vi "close.vi"(8 "error in":errorcluster, 11 "Scan Engine runtime in":refnum<class "Scan Engine runtime.lvclass">) -> (0 "error out":errorcluster)   [LabVIEW 2015, in "Scan Engine runtime.lvclass"]
doc: "Provides an interface for terminating a module instance. While this interface performs no operations, a child should close and deallocate any open references or memory."
uses:
  Scan Engine runtime.lvclass
  Scan Engine runtime.lvclass/Scan Engine runtime.ctl
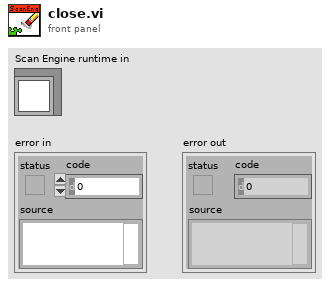
[diagram p1: front panel]
types:
  T1 = typedef "Scan Engine runtime.lvclass/Index Map.ctl" = cluster{"data type":T2, "variable ref":refnum<k21>, "index":i32, "IO Var":bool, "module_index":i32}
  T2 = typedef "tag bus.lvlib/tag descriptor.lvclass/Data Type.ctl" = enum16{"Double", "Single", "I64", "I32", "I16", "I8", "U64", "U32", "U16", "U8", "Boolean", "String", "Array of Double", "Array of Single", "Array of I64", "Array of I32", "Array of I16", "Array of I8", "Array of U64", "Array of U32", "Array of U16", "Array of U8", "Array of Boolean", "Array of String"}
  T3 = typedef "Scan Engine runtime.lvclass/IO_index_map.ctl" = cluster{"module_ref":refnum<k21>, "data type":T2, "IO_variable_info":T1[], "IO_module_index_array":i32[], "IO_table_index":i32[], "IO_table_index_ordered":i32[], "use_scanned_methods":bool}
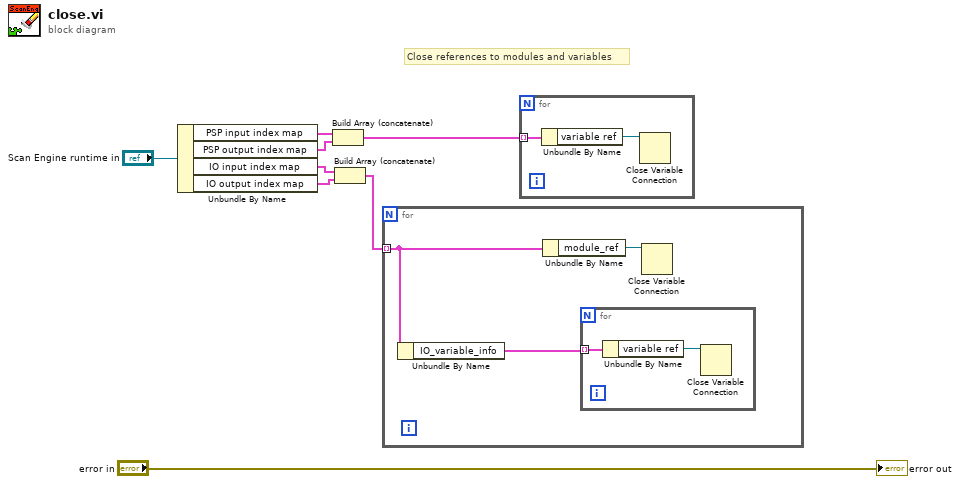
[diagram p0: block diagram]
diagram:
  # "Close references to modules and variables"
  n1 = Unbundle By Name("Scan Engine runtime in") -> ("PSP input index map"=w6:T1[], "PSP output index map"=w5:T1[], "IO input index map"=w3:T3[], "IO output index map"=w2:T3[])
  n2 = Build Array (concatenate)(w6, w5) -> (w4:T1[])
  n3 = Build Array (concatenate)(w3, w2) -> (w1:T3[])
  n4 = for {
    tunnel: w1 -> [w10] mode=indexing
    n5 = Unbundle By Name(w10) -> ("IO_variable_info"=w9:T1[])
    n6 = Unbundle By Name(w10) -> ("module_ref"=w11:refnum<k21>)
    n7 = for {
      tunnel: w9 -> [w13] mode=indexing
      n8 = Unbundle By Name(w13) -> ("variable ref"=w12:refnum<k21>)
      n9 = Close Variable Connection(11:w12) -> ()  [unwired: 1 in, 1 out]
    }
    n10 = Close Variable Connection(11:w11) -> ()  [unwired: 1 in, 1 out]
  }
  n11 = for {
    tunnel: w4 -> [w15] mode=indexing
    n12 = Unbundle By Name(w15) -> ("variable ref"=w14:refnum<k21>)
    n13 = Close Variable Connection(11:w14) -> ()  [unwired: 1 in, 1 out]
  }
  "error out" <- "error in"
